vi "Apply Opacity.vi"(7 "% (100)":u8=100, 9 "Bottom":picture, 11 "Top":picture) -> (3 "new picture":picture)   [LabVIEW 2020, in "lv_icon.lvlib"]
doc: "Merge two glyphs and apply a certain opacity to the Top glyph.s"
uses:
  lv_icon.lvlib
  <vilib>/picture/picture.llb/Draw True-Color Pixmap.vi
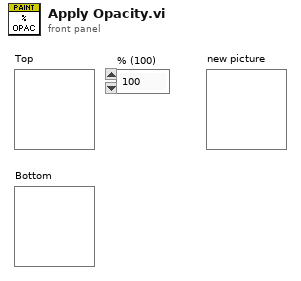
[diagram p1: front panel]
types:
  T1 = cluster{"left":i16, "top":i16, "right":i16, "bottom":i16}
  T2 = typedef "imagedata.ctl" = cluster{"image type":i32, "image depth":i32, "image":u8[], "mask":u8[], "colors":u32[], "Rectangle":cluster{"left":i16, "top":i16, "right":i16, "bottom":i16}}
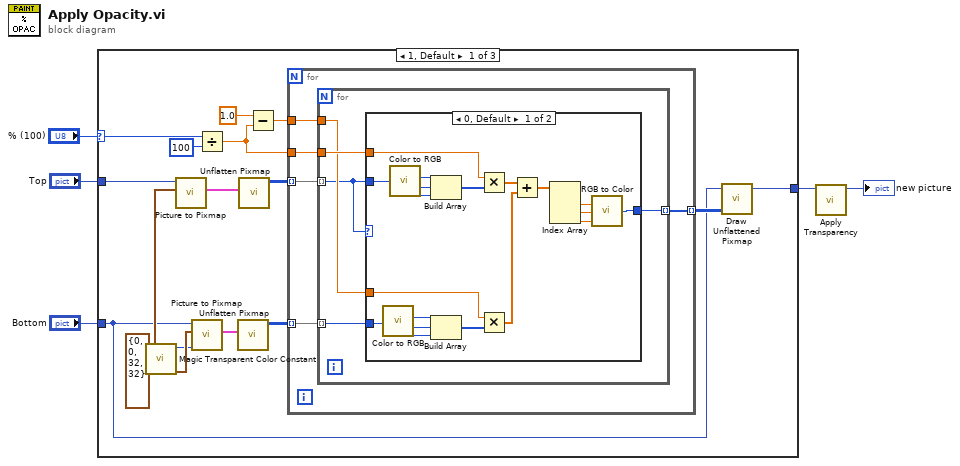
[diagram p0: block diagram]
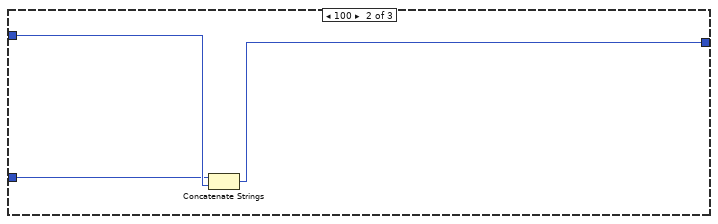
[diagram p3: hidden frame]
diagram:
  n1 = case shown="1, Default" "% (100)" {
    selector: "% (100)" -> [w9 _ _]
    tunnel: [w7 w51 w54] -> w2
    tunnel: "Bottom" -> [w8 w52 w54]
    tunnel: "Top" -> [w14 w53 _]
    frame 1, Default {
      w12 = T1 {"left"=0, "top"=0, "right"=32, "bottom"=32} ("rect")
      n2 = call "Magic Transparent Color Constant.vi"() -> ("Magic transparent color constant"=w6:u32)  [unwired: 11 out]
      n3 = call <vilib>:"Picture to Pixmap.vi"("rect"=w12, "picture"=w14) -> ("image data"=w13:T2)  [unwired: 2 in, 7 out]
      n4 = call <vilib>:"Picture to Pixmap.vi"("Background Color"=w6, "rect"=w12, "picture"=w8) -> ("image data"=w15:T2)  [unwired: 1 in, 7 out]
      n5 = Divide(x=w9, y=u8 100) -> (x/y=w10:dbl)
      n6 = call <vilib>:"Unflatten Pixmap.vi"("image data"=w15) -> ("24-bit pixmap"=w17:u32[][])  [unwired: 10 out]
      n7 = call <vilib>:"Unflatten Pixmap.vi"("image data"=w13) -> ("24-bit pixmap"=w16:u32[][])  [unwired: 10 out]
      n8 = Subtract(x=1.0, y=w10) -> (x-y=w18:dbl)
      n9 = for {
        tunnel: w16 -> [w25] mode=indexing
        tunnel: w10 -> [w24]
        tunnel: [w23] -> w20 mode=indexing
        tunnel: w18 -> [w22]
        tunnel: w17 -> [w21] mode=indexing
        n10 = for {
          tunnel: w25 -> [w26] mode=indexing
          tunnel: w24 -> [w30]
          tunnel: [w29] -> w23 mode=indexing
          tunnel: w22 -> [w27]
          tunnel: w21 -> [w28] mode=indexing
          n11 = case shown="0, Default" w26 {
            tunnel: w30 -> [w45 _]
            tunnel: [w41 w50] -> w29
            tunnel: w28 -> [w36 w50]
            tunnel: w27 -> [w35 _]
            tunnel: w26 -> [w31 _]
            frame 0, Default {
              n12 = call <vilib>:"Color to RGB.vi"("Color"=w36) -> ("R"=w39:u8, "G"=w38:u8, "B"=w37:u8)  [unwired: 1 out]
              n13 = call <vilib>:"Color to RGB.vi"("Color"=w31) -> ("R"=w47:u8, "G"=w48:u8, "B"=w49:u8)  [unwired: 1 out]
              n14 = Build Array(w47, w48, w49) -> (w46:u8[])
              n15 = Build Array(w39, w38, w37) -> (w40:u8[])
              n16 = Multiply(x=w45, y=w46) -> (x*y=w34:dbl[])
              n17 = Multiply(x=w35, y=w40) -> (x*y=w33:dbl[])
              n18 = Add(x=w34, y=w33) -> (x+y=w32:dbl[])
              n19 = Index Array(array=w32) -> (element #1=w43:dbl, element #2=w44:dbl, element #3=w42:dbl)  [unwired: 3 in]
              n20 = call <vilib>:"RGB to Color.vi"("B"=w42, "G"=w44, "R"=w43) -> ("Color"=w41:u32)
            }
            frame 16777215 {
              # "True White color"
            }
          }
        }
      }
      n21 = call-poly <vilib>:"Draw Unflattened Pixmap.vi"("picture"=w8, "data (RGB format)"=w20) -> ("new picture"=w7:picture)  [unwired: 2 in, 5 out]
    }
    frame 100 {
      n22 = Concatenate Strings(w52, w53) -> (w51:picture)
    }
    frame 0 {
    }
  }
  n23 = call "Apply Transparency.vi"("in"=w2) -> ("out"=→"new picture":picture)  [unwired: 10 in]
